vi "lookup_node_predecessors_by_id.vi"(10 "node-id":refnum<class "ID.lvclass">, 11 "Graph in":refnum<class "DiGraph.lvclass">) -> (1 "predecessors":set{refnum<class "ID.lvclass">}(c389), 2 "node not found?":bool)   [LabVIEW 2020, in "graph.lvlib" / "DiGraph.lvclass"]
uses:
  DiGraph.lvclass
  DiGraph.lvclass/DiGraph.ctl
  ID/ID.lvclass
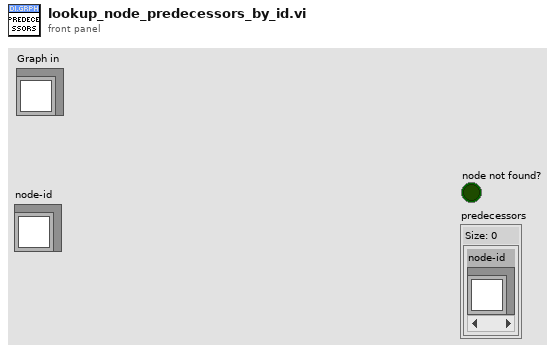
[diagram p1: front panel]
types:
  T1 = map{refnum<class "ID.lvclass">, set{refnum<class "ID.lvclass">}}
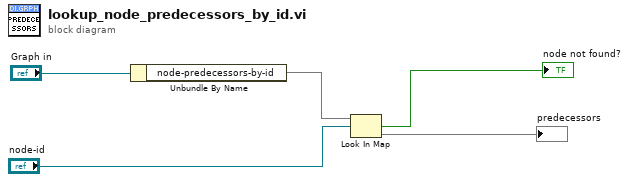
[diagram p0: block diagram]
diagram:
  n1 = Unbundle By Name("Graph in") -> ("node-predecessors-by-id"=w1:T1)
  n2 = Look In Map(map=w1, key="node-id") -> (key not found?=→"node not found?":bool, value=→"predecessors":set{refnum<class "ID.lvclass">})  [unwired: 1 in]
